vi "Check Action.vi"(6 "HRS Time":dbl, 7 "Values In":dbl[](array[numeric]), 8 "error in (no error)":errorcluster, 11 "Valve in":refnum<class "HitAndHoldControl.lvclass">) -> (0 "error out":errorcluster, 2 "Actions":T1[](array[typedef]), 3 "Valve out":refnum<class "HitAndHoldControl.lvclass">, 5 "Values":dbl[](array[numeric]))   [LabVIEW 2020, in "VolatusControl.lvlib" / "HitAndHoldControl.lvclass"]
uses:
  HitAndHoldControl.lvclass
  Control Action.ctl
  Volatus/MessageQ/MessageQ.lvclass
  HitAndHoldControl.lvclass/HitAndHoldControl.ctl
  HitAndHold State.ctl
  messages/CmdAnalog/Data.ctl
  Volatus/MessageQ/MessageQ.lvclass/MessageQ.ctl
  messages/CmdAnalog/CmdAnalog.lvlib
  VolatusControl.lvlib
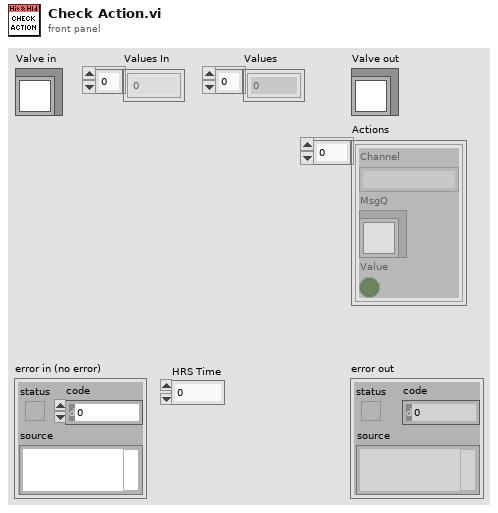
[diagram p1: front panel]
types:
  T1 = typedef "VolatusControl.lvlib/Control Action.ctl" = cluster{"Channel":string, "MsgQ":refnum<class "MessageQ.lvclass">, "Value":bool}
  T2 = typedef "VolatusControl.lvlib/HitAndHoldControl.lvclass/HitAndHold State.ctl" = enum16{"Idle", "Hit", "Dwell", "Hold", "Off"}
  T3 = typedef "CmdAnalog.lvlib/Data.ctl" = cluster{"channel":string, "value":dbl}
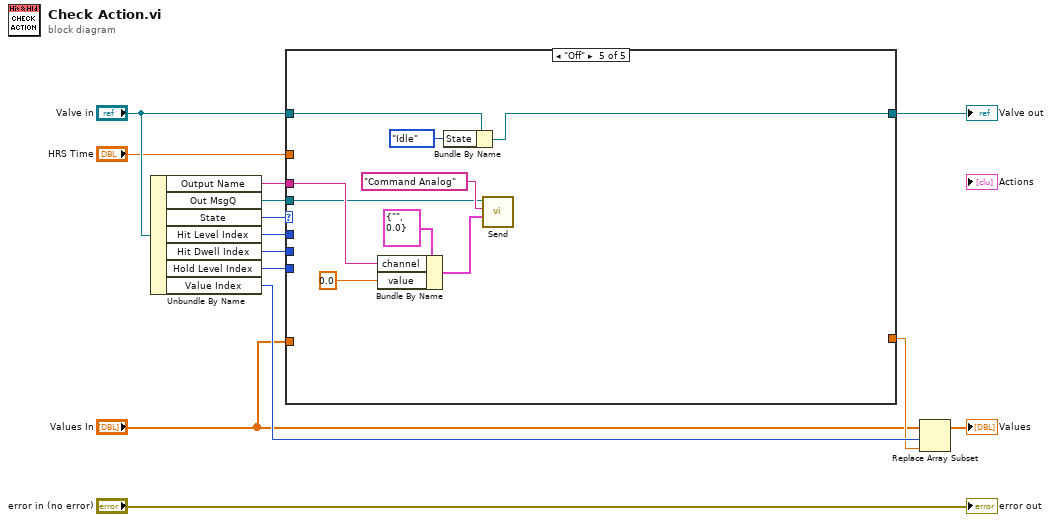
[diagram p0: block diagram]
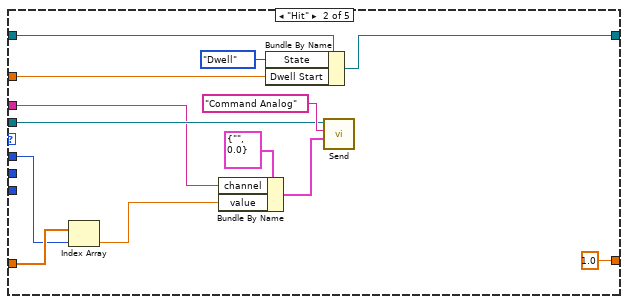
[diagram p3: hidden frame]
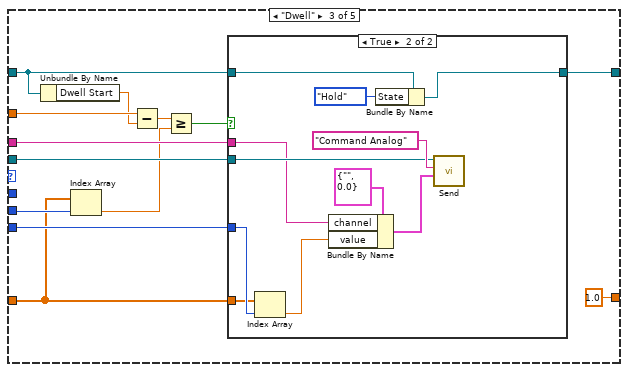
[diagram p4: hidden frame]
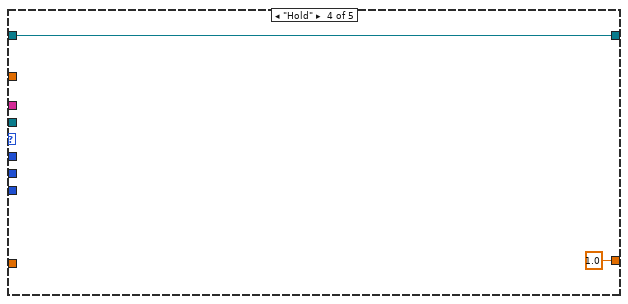
[diagram p6: hidden frame]
diagram:
  n1 = Unbundle By Name("Valve in") -> ("Output Name"=w4:string, "Out MsgQ"=w11:refnum<class "MessageQ.lvclass">, "State"=w12:T2, "Hit Level Index"=w10:i32, "Hit Dwell Index"=w9:i32, "Hold Level Index"=w8:i32, "Value Index"=w6:i32)
  n2 = case shown="\"Off\"" w12 {
    tunnel: "Valve in" -> [w15 w27 w39 w54 w58]
    tunnel: w11 -> [_ w20 w37 _ w60]
    tunnel: w10 -> [_ w17 _ _ _]
    tunnel: w9 -> [_ _ w40 _ _]
    tunnel: w8 -> [_ _ w35 _ _]
    tunnel: [_ 1.0 1.0 1.0 _] -> w5
    tunnel: w4 -> [_ w19 w36 _ w61]
    tunnel: "Values In" -> [_ w18 w34 _ _]
    tunnel: "HRS Time" -> [_ w24 w33 _ _]
    tunnel: [w15 w26 w38 w54 w57] -> w1
    frame "Idle" {
    }
    frame "Hit" {
      n3 = Index Array(array=w18, index=w17) -> (element=w16:dbl)
      n4 = Bundle By Name(cluster=T3 {"channel"="", "value"=0.0} ("CmdAnalog"), "channel"=w19, "value"=w16) -> (w22:T3)
      n5 = Bundle By Name(cluster=w27, "State"=HitAndHold_State."Dwell", "Dwell Start"=w24) -> (w26:refnum<class "HitAndHoldControl.lvclass">)
      n6 = call "Send.vi"("Data"=w22, "ID"="Command Analog", "MessageQ in"=w20) -> ()  [unwired: 7 in, 2 out]
    }
    frame "Dwell" {
      n7 = Unbundle By Name(w39) -> ("Dwell Start"=w32:dbl)
      n8 = Index Array(array=w34, index=w40) -> (element=w30:dbl)
      n9 = Subtract(x=w33, y=w32) -> (x-y=w31:dbl)
      n10 = Greater Or Equal?(x=w31, y=w30) -> (x >= y?=w29:bool)
      n11 = case shown="True" w29 {
        tunnel: w39 -> [w42 w53]
        tunnel: [w42 w52] -> w38
        tunnel: w37 -> [_ w45]
        tunnel: w36 -> [_ w44]
        tunnel: w35 -> [_ w50]
        tunnel: w34 -> [_ w49]
        frame False {
        }
        frame True {
          n12 = Index Array(array=w49, index=w50) -> (element=w43:dbl)
          n13 = Bundle By Name(cluster=T3 {"channel"="", "value"=0.0} ("CmdAnalog"), "channel"=w44, "value"=w43) -> (w47:T3)
          n14 = Bundle By Name(cluster=w53, "State"=HitAndHold_State."Hold") -> (w52:refnum<class "HitAndHoldControl.lvclass">)
          n15 = call "Send.vi"("Data"=w47, "ID"="Command Analog", "MessageQ in"=w45) -> ()  [unwired: 7 in, 2 out]
        }
      }
    }
    frame "Hold" {
    }
    frame "Off" {
      n16 = Bundle By Name(cluster=T3 {"channel"="", "value"=0.0} ("CmdAnalog"), "channel"=w61, "value"=0.0) -> (w63:T3)
      n17 = Bundle By Name(cluster=w58, "State"=HitAndHold_State."Idle") -> (w57:refnum<class "HitAndHoldControl.lvclass">)
      n18 = call "Send.vi"("Data"=w63, "ID"="Command Analog", "MessageQ in"=w60) -> ()  [unwired: 7 in, 2 out]
    }
  }
  "Valve out" <- w1
  n19 = Replace Array Subset(array="Values In", new element=w5, index=w6) -> (→"Values":dbl[])
  "error out" <- "error in (no error)"
